vi "DAC Run.vi"(8 "error in":errorcluster, 11 "DAC Keller Diff P 23X in":refnum<class "DAC Keller Diff P 23X.lvclass">) -> (0 "error out":errorcluster, 3 "DAC Keller Diff P 23X out":refnum<class "DAC Keller Diff P 23X.lvclass">)   [LabVIEW 2019, in "DAC.lvlib" / "DAC Keller Diff P 23X.lvclass"]
uses:
  DAC Keller Diff P 23X.lvclass
  C:/Users/krio/Documents/LV_Projects/test-stand/App/DAC/DAC.lvclass
  DAC.lvclass/DAC.ctl
  Results/Results Method.ctl
  Results/DeepU Results/DeepU Results.lvclass
  DAC Keller Diff P 23X.lvclass/DAC Keller Diff P 23X.ctl
  <vilib>/Platform/TimedLoop/XDataNode/timing_clust.ctl
  <vilib>/Platform/TimedLoop/XDataNode/nitl_modes.ctl
  <vilib>/Platform/TimedLoop/XDataNode/wakeup.ctl
  <instrlib>/_KELLER RS485 Library/Public/Type Definitions/Channel.ctl
  <vilib>/platform/TimedLoop/XDataNode/XDataNode.xnode
  DAC.lvclass
  Results/Results.lvlib
  <instrlib>/_KELLER RS485 Library/KELLER RS485 Library.lvlib
  <vilib>/Platform/TimedLoop/XDataNode/XDNodeRunTimeDep.lvlib
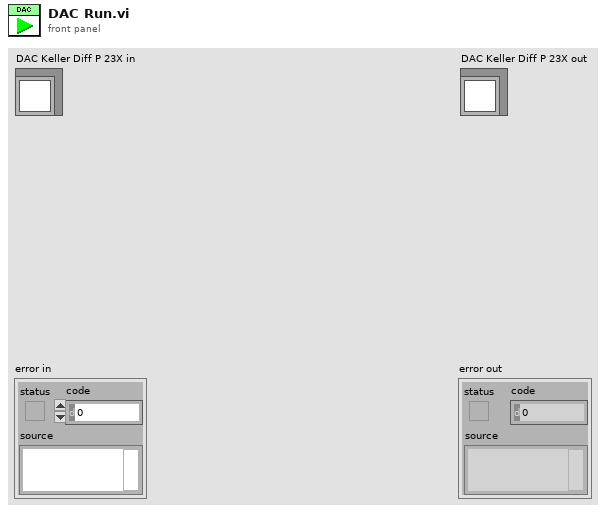
[diagram p1: front panel]
types:
  T1 = typedef "Results.lvlib/Results Method.ctl" = enum16{"Get", "Set"}
  T2 = typedef "KELLER RS485 Library.lvlib/Channel.ctl" = enum16{"CH0", "P1", "P2", "T", "TOB1", "TOB2", "TE", "CH7", "CH8", "CH9", "ConTc", "ConRaw", "CH12"}
  T3 = typedef "XDNodeRunTimeDep.lvlib/timing_clust.ctl" = cluster{"Expected End [f-1]":u64, "Actual End [f-1]":u64, "Finished Late? [f-1]":bool, "Expected End [i-1]":u64, "Actual End [i-1]":u64, "Finished Late? [i-1]":bool, "Expected Start [i]":u64, "Actual Start [i]":u64, "Expected Start [f]":u64, "Actual Start [f]":u64, "Source Name":string, "Structure Name":string, "Period":i64, "Deadline":i64, "Offset":i64, "Start":i64, "Priority":i32, "Timeout":i32, "Mode":T4, "Wakeup Reason":T5, "Error":errorcluster, "Source Type":string, "Secondary Source Type":string, "Global End Time":u64, "Global Start Time":u64, "Frame Duration":u64, "Iteration Duration":u64, "Assigned CPU":i32, "I/O Scan Engine Mode":u32}
  T4 = typedef "XDNodeRunTimeDep.lvlib/nitl_modes.ctl" = enum32{"No Change", "Process missed periods, maintain original phase", "Discard missed periods, maintain original phase", "Process missed periods, ignore original phase", "Discard missed periods, ignore original phase"}
  T5 = typedef "XDNodeRunTimeDep.lvlib/wakeup.ctl" = enum32{"Normal", "Aborted", "Asynchronous wakeup", "Timing source error", "Timed loop error", "Timeout"}
  T6 = typedef "KELLER RS485 Library.lvlib/Bus.ctl" = cluster{"VISA":refnum<visa-resource-name>, "Baud Rate ":T7, "Timeout":u32, "Echo?":bool, "Wait before transmit":u32}
  T7 = typedef "KELLER RS485 Library.lvlib/Baud Rate.ctl" = enum16{"9600bd", "115200bd"}
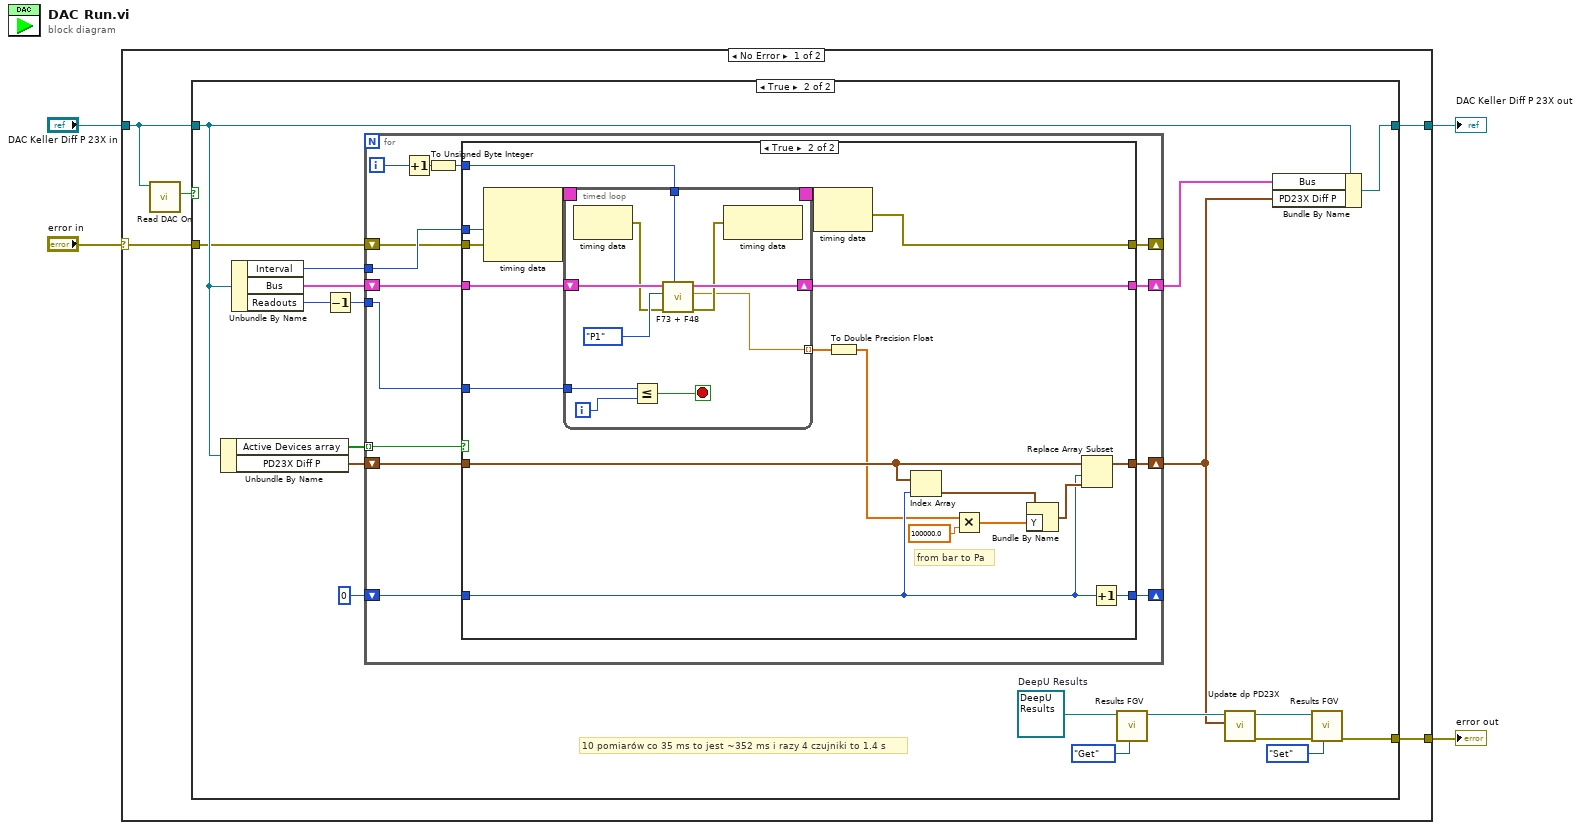
[diagram p0: block diagram]
diagram:
  n1 = case shown="No Error" "error in" {
    selector: "error in" -> [w7 w90]
    tunnel: [w6 w90] -> w2
    tunnel: [w8 w89] -> w1
    tunnel: "DAC Keller Diff P 23X in" -> [w5 w89]
    frame No Error {
      n2 = call "Read DAC On.vi"("DAC in"=w5) -> ("DAC On"=w9:bool)  [unwired: 8 in, 2 out]
      n3 = case shown="True" w9 {
        tunnel: w5 -> [w11 w17]
        tunnel: [w11 w23] -> w8
        tunnel: w7 -> [w10 w13]
        tunnel: [w10 w27] -> w6
        frame False {
        }
        frame True {
          w30 = refnum<class "DeepU Results.lvclass"> refnum  # DeepU Results
          # "10 pomiarów co 35 ms to jest ~352 ms i razy 4 czujniki to 1.4 s"
          n4 = Unbundle By Name(w17) -> ("Active Devices array"=w22:bool[], "PD23X Diff P"=w21:waveform(dbl)[])
          n5 = Unbundle By Name(w17) -> ("Interval"=w15:i64, "Bus"=w16:T6, "Readouts"=w14:i32)
          n6 = Decrement(x=w14) -> (x-1=w12:i32)
          n7 = for {
            tunnel: w22 -> [w41] mode=indexing
            shift-right: [w39] -> w18
            shift-left: w21 -> [w40]
            shift-right: [w38] -> w20
            shift-left: w16 -> [w43]
            shift-right: [w35] -> _
            shift-left: 0 -> [w36]
            tunnel: w15 -> [w34]
            tunnel: w12 -> [w33]
            shift-right: [w31] -> _
            shift-left: w13 -> [w32]
            i -> [w37]
            n8 = Increment(x=w37) -> (x+1=w44:i32)
            n9 = To Unsigned Byte Integer(number=w44) -> (unsigned 8bit integer=w42:u8)
            n10 = case shown="True" w41 {
              tunnel: w43 -> [w47 w67]
              tunnel: w42 -> [_ w66]
              tunnel: w40 -> [w48 w61]
              tunnel: [w48 w65] -> w39
              tunnel: [w47 w64] -> w38
              tunnel: w36 -> [w46 w59]
              tunnel: [w46 w62] -> w35
              tunnel: w34 -> [_ w55]
              tunnel: w33 -> [_ w54]
              tunnel: w32 -> [w45 w53]
              tunnel: [w45 w52] -> w31
              frame False {
              }
              frame True {
                # "from bar to Pa"
                n11 = node-c288(w55, w53) -> (w57:T3)  [unwired: 1 in]
                n12 = timed-loop {
                  timing: w57 -> [_]
                  timing-out: [_] -> w56
                  tunnel: w66 -> [w76]
                  tunnel: [w68] -> w51 mode=indexing
                  shift-right: [w75] -> w64
                  shift-left: w67 -> [w77]
                  tunnel: w54 -> [w73]
                  i -> [w72]
                  stop <- w71 stop-if-true
                  n13 = node-c288() -> (w70:errorcluster)  [unwired: 1 in]
                  n14 = Less Or Equal?(x=w73, y=w72) -> (x <= y?=w71:bool)
                  n15 = call <instrlib>:"F73 + F48.vi"("Address (250)"=w76, "error in (no error)"=w70, "Channel (P1)"=Channel."P1", "Bus in"=w77) -> ("error out"=w69:errorcluster, "Value as Single"=w68:sgl, "Bus out"=w75:T6)  [unwired: 3 in, 2 out]
                  n16 = node-c288(w69) -> ()  [unwired: 1 out]
                }
                n17 = node-c288(w56) -> (w52:errorcluster)
                n18 = To Double Precision Float(number=w51) -> (double precision float=w49:dbl[])
                n19 = Index Array(array=w61, index=w59) -> (element=w60:waveform(dbl))
                n20 = Multiply(x=w49, y=100000.0 ("x")) -> (x*y=w50:dbl[])
                n21 = Bundle By Name(cluster=w60, "Y"=w50) -> (w63:waveform(dbl))
                n22 = Replace Array Subset(array=w61, new element=w63, index=w59) -> (w65:waveform(dbl)[])
                n23 = Increment(x=w59) -> (x+1=w62:i32)
              }
            }
          }
          n24 = call-dynamic "Results FGV.vi"("Method"=Results_Method."Get", "DeepU Results in"=w30) -> ("DeepU Results out"=w25:refnum<class "DeepU Results.lvclass">)  [unwired: 8 in, 1 out]
          n25 = call "Update dp PD23X.vi"("dp PD-23X"=w18, "DeepU Results in"=w25) -> ("error out"=w26:errorcluster, "DeepU Results out"=w24:refnum<class "DeepU Results.lvclass">)  [unwired: 8 in]
          n26 = Bundle By Name(cluster=w17, "Bus"=w20, "PD23X Diff P"=w18) -> (w23:refnum<class "DAC Keller Diff P 23X.lvclass">)
          n27 = call-dynamic "Results FGV.vi"("Method"=Results_Method."Set", "error in"=w26, "DeepU Results in"=w24) -> ("error out"=w27:errorcluster)  [unwired: 7 in, 1 out]
        }
      }
    }
    frame Error {
    }
  }
  "error out" <- w2
  "DAC Keller Diff P 23X out" <- w1
